vi "Channel Read Write.vi"(11 "plugin gRPC address":string="localhost:51930") -> ()   [LabVIEW 2021, in "CAN_Reader_NIXNET_Test_Helpers.lvlib"]
uses:
  CAN_Reader_NIXNET_Test_Helpers.lvlib
  <vilib>/CIF Foundation/CIF Core/CIFCore/Common/Typedef/gRPC Reported Plugin Status.ctl
  <vilib>/CIF Foundation/CIF Core/CIFCore/Common/Typedef/Plugin State.ctl
  <vilib>/CIF Foundation/CIF Core/CIFCore/Common/Typedef/Timing Statistics.ctl
  <vilib>/CIF Foundation/CIF Core/CIFCore/Common/Typedef/Timing Stats Base.ctl
  <vilib>/CIF Foundation/CIF Core/CIFCore/Common/Typedef/FIFO Statistics.ctl
  <vilib>/CIF Foundation/CIF Core/CIFCore/Common/Typedef/Simple Error.ctl
  <vilib>/CIF Foundation/CIF Core/CIFCore/Common/Typedef/Monitor Doubles.ctl
  <vilib>/CIF Foundation/CIF Core/CIFCore/Common/Typedef/Monitor U64.ctl
  <vilib>/CIF Foundation/CIF Core/CIFCore/Common/Typedef/Monitor I64.ctl
  <vilib>/CIF Foundation/CIF Channels Core/ChannelCommon/typedef/FIFO Header.ctl
  <vilib>/xnet/xnet.llb/XNET Frame CAN.ctl
  <vilib>/xnet/xnet.llb/XNET Frame Type CAN.ctl
  Common/Typedef/Channels.ctl
  <vilib>/CIF Foundation/CIF Core/CIFCore/Class/CIFCorePlugin.lvclass/CIFCorePlugin.ctl
  <vilib>/CIF Foundation/CIF Utilities/Statistics/I64/Stats_I64_CIF_U.lvclass/Stats_I64_CIF_U.ctl
  <vilib>/CIF Foundation/CIF XNET CAN RW/XNET CAN RW.lvclass
  C:/Program Files/National Instruments/LabVIEW 2021/vi.lib/CIF Foundation/CIF CAN RW Core/CAN_RW_CORE.lvclass
  <vilib>/CIF Foundation/CIF CAN RW Core/CAN_RW_CORE.lvclass/CAN_RW_CORE.ctl
  <vilib>/CIF Foundation/CIF PCAP Parse and Build/pcap_Parse_Build_CIF.lvclass/pcap_Parse_Build_CIF.ctl
  <vilib>/CIF Foundation/CIF Core/CIFCore/Class/Benchmarking/Benchmark FIFO Read.vi
  <vilib>/CIF Foundation/CIF XNET CAN RW/Utilities/Header Cluster to XNET CAN.vi
  <vilib>/CIF Foundation/CIF PCAP Parse and Build/Parse/Parse Packet Header.vi
  <vilib>/CIF Foundation/CIF PCAP Parse and Build/Parse/Unflatten Socket CAN Header.vi
  <vilib>/CIF Foundation/CIF PCAP Parse and Build/Utilities/Get Data Segment.vi
  <vilib>/CIF Foundation/CIF PCAP Parse and Build/Data Accessors/Read Offset.vi
  <vilib>/CIF Foundation/CIF CAN RW Core/Utilities/Filter Packets.vi
  <vilib>/CIF Foundation/CIF CAN RW Core/Accessors/Read pcap class.vi
  <vilib>/CIF Foundation/CIF CAN RW Core/Accessors/Write pcap class.vi
  <vilib>/CIF Foundation/CIF PCAP Parse and Build/Data Accessors/Write Offset.vi
  <vilib>/CIF Foundation/CIF Utilities/Statistics/I64/X1 minus X0.vi
  <vilib>/CIF Foundation/CIF Utilities/Time/System Time/Get System Time.vi
  <vilib>/CIF Foundation/CIF Utilities/Time/System Time/TAI Time to LabVIEW Time.vi
  <vilib>/CIF Foundation/CIF PCAP Parse and Build/Parse/Unflatten Packet Header.vi
  <vilib>/CIF Foundation/CIF Utilities/DataTypes/Flatten Unflatten/Unflatten U32.vi
  <vilib>/CIF Foundation/CIF PCAP Parse and Build/Utilities/Add Error.vi
  <vilib>/CIF Foundation/CIF Utilities/Statistics/I64/X1 minus X0.vi/dfabcf33-0dbc-4041-80a5-3dc0c86d2989.vi
  <vilib>/CIF Foundation/CIF Utilities/Errors/Append Error Location.vi
  <vilib>/CIF Foundation/CIF Utilities/Statistics/I64/X1 minus X0.vi/dfabcf33-0dbc-4041-80a5-3dc0c86d2989.vi/9eb60a9a-770f-4d2d-8b3f-8465c267ecc9.vi
  <vilib>/gRPC/LabVIEW gRPC Library/Client API/Close Client.vi
  <vilib>/CIF Foundation/CIF PCAP Parse and Build/pcap_Parse_Build_CIF.lvclass
  <vilib>/CIF Foundation/CIF Channels Core/CIFChannels/CIFChannels.lvclass
  <vilib>/CIF Foundation/CIF Core/CIFCore/Grpc/CIFCoreWrapper/CIFCoreWrapper.lvlib
  <vilib>/CIF Foundation/CIF Core/CIFCore/Class/CIFCorePlugin.lvclass
  Common/CAN_Reader_NIXNET_Common.lvlib
  Grpc/CAN_Reader_NIXNET_wrapper/CAN_Reader_NIXNET_Wrapper.lvlib
  <vilib>/CIF Foundation/CIF Utilities/DataTypes/DataTypes_CIF_U.lvlib
  <vilib>/CIF Foundation/CIF Utilities/Time/Time_CIF_U.lvlib
  <vilib>/CIF Foundation/CIF Core/CIFCore/Common/CIFCoreCommon.lvlib
  <vilib>/CIF Foundation/CIF Channels Core/ChannelCommon/ChannelCommon.lvlib
panel:
  out "x-y":i64 format="%.5e"
  out "Raw Bytes":string
  out "XNET CAN Data":T1[](array[typedef]) {"payload" format="%x"; "timestamp" format="%<%.7X\n%x>T"; "type" items=["CAN Data"=0, "CAN Remote"=1, "CAN Bus Error"=2, "CAN 2.0 Data"=8, "CAN FD Data"=16, "CAN FD+BRS Data"=24, "J1939 Data"=192, "Delay"=224, "Log Trigger"=225, "Start Trigger"=226]; "identifier" format="%x"}
  out "Header":T3
  out "Node Status":T4 {"Monitor Doubles"."4" format="%#_9g"; "Monitor Doubles"."3" format="%#_9g"; "Monitor Doubles"."2" format="%#_9g"; "Monitor Doubles"."1" format="%#_9g"; "Timing Statistics (us)"."Period"."Avg" format="%_6g"}
  in  "EXIT":bool
  in  "Unload":bool
  out "error out":errorcluster
  # "Update plugin gRPC address including gRPC port and run on same target as the plugin code. \nExit will stop this VI.\nUnload will stop this VI and unload the plugin."
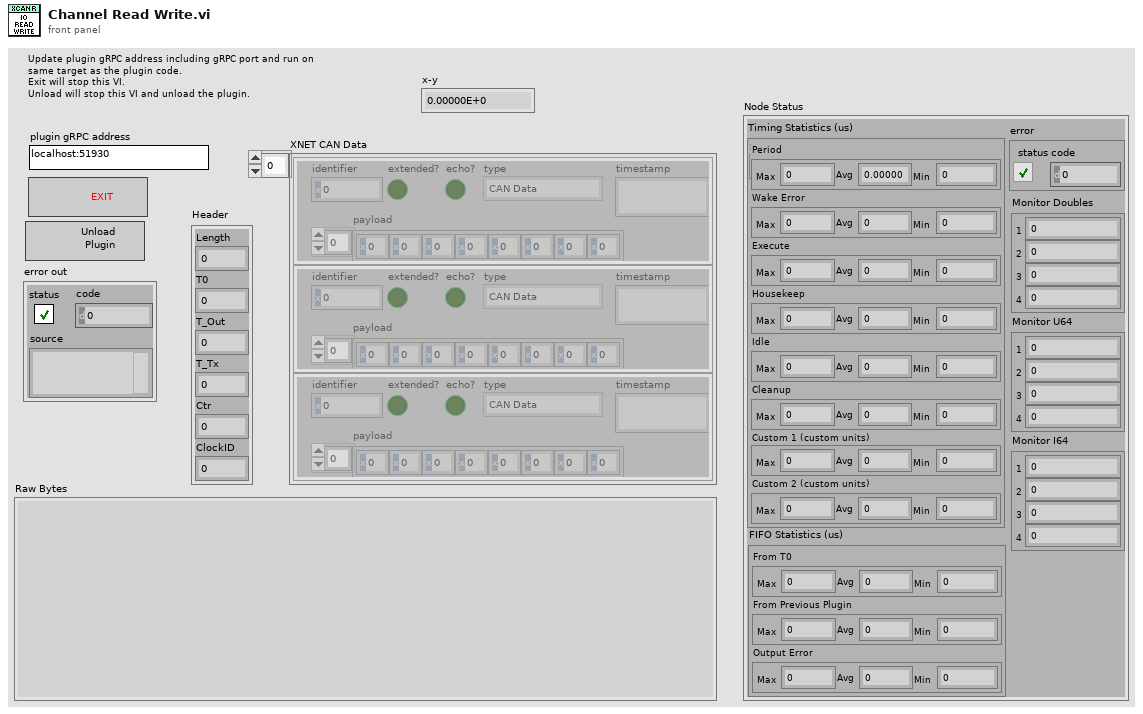
[diagram p1: front panel]
types:
  T1 = typedef "XNET Frame CAN.ctl" = cluster{"timestamp":timestamp, "payload":u8[], "identifier":u32, "type":T2, "extended?":bool, "echo?":bool}
  T2 = typedef "XNET Frame Type CAN.ctl" = u8
  T3 = typedef "ChannelCommon.lvlib/FIFO Header.ctl" = cluster{"Length":u64, "T0":i64, "T_Out":i64, "T_Tx":i64, "Ctr":u64, "ClockID":u8}
  T4 = typedef "CIFCoreCommon.lvlib/gRPC Reported Plugin Status.ctl" = cluster{"State":T5, "Timing Statistics (us)":T6, "FIFO Statistics (us)":T8, "error":T9, "Monitor Doubles":T10, "Monitor U64":T11, "Monitor I64":T12}
  T5 = typedef "CIFCoreCommon.lvlib/Plugin State.ctl" = enum32{"Null", "Creating", "Listening", "Running", "CleaningUp", "Destroying"}
  T6 = typedef "CIFCoreCommon.lvlib/Timing Statistics.ctl" = cluster{"Period":T7, "Wake Error":T7, "Execute":T7, "Housekeep":T7, "Idle":T7, "Cleanup":T7, "Custom 1 (custom units)":T7, "Custom 2 (custom units)":T7}
  T7 = typedef "CIFCoreCommon.lvlib/Timing Stats Base.ctl" = cluster{"Max":i64, "Avg":dbl, "Min":i64}
  T8 = typedef "CIFCoreCommon.lvlib/FIFO Statistics.ctl" = cluster{"From T0":T7, "From Previous Plugin":T7, "Output Error":T7}
  T9 = typedef "CIFCoreCommon.lvlib/Simple Error.ctl" = cluster{"status":bool, "code":i32}
  T10 = typedef "CIFCoreCommon.lvlib/Monitor Doubles.ctl" = cluster{"1":dbl, "2":dbl, "3":dbl, "4":dbl}
  T11 = typedef "CIFCoreCommon.lvlib/Monitor U64.ctl" = cluster{"1":u64, "2":u64, "3":u64, "4":u64}
  T12 = typedef "CIFCoreCommon.lvlib/Monitor I64.ctl" = cluster{"1":i64, "2":i64, "3":i64, "4":i64}
  T13 = typedef "grpc-lvsupport-release.lvlib/grpcId.ctl" = u64
  T14 = typedef "CIFCoreChannel_client.lvlib/cif_channelcore_Channel.ctl" = cluster{"name":string, "direction":T15, "type":string, "custom_config":u8[], "connected":bool, "connected_name":string, "forced":bool, "channel_pattern":T16}
  T15 = typedef "CIFCoreChannel_client.lvlib/cif_channelcore_Direction.ctl" = enum32{"PUBLISHER", "SUBSCRIBER"}
  T16 = typedef "CIFCoreChannel_client.lvlib/cif_channelcore_PATTERN.ctl" = enum32{"UNKNOWN", "TAG", "FIFO", "MULTIFIFO", "BACKPRESSUREFIFO"}
  T17 = typedef "CAN_Reader_NIXNET_Common.lvlib/Channels.ctl" = enum16{"CAN_Frames"}
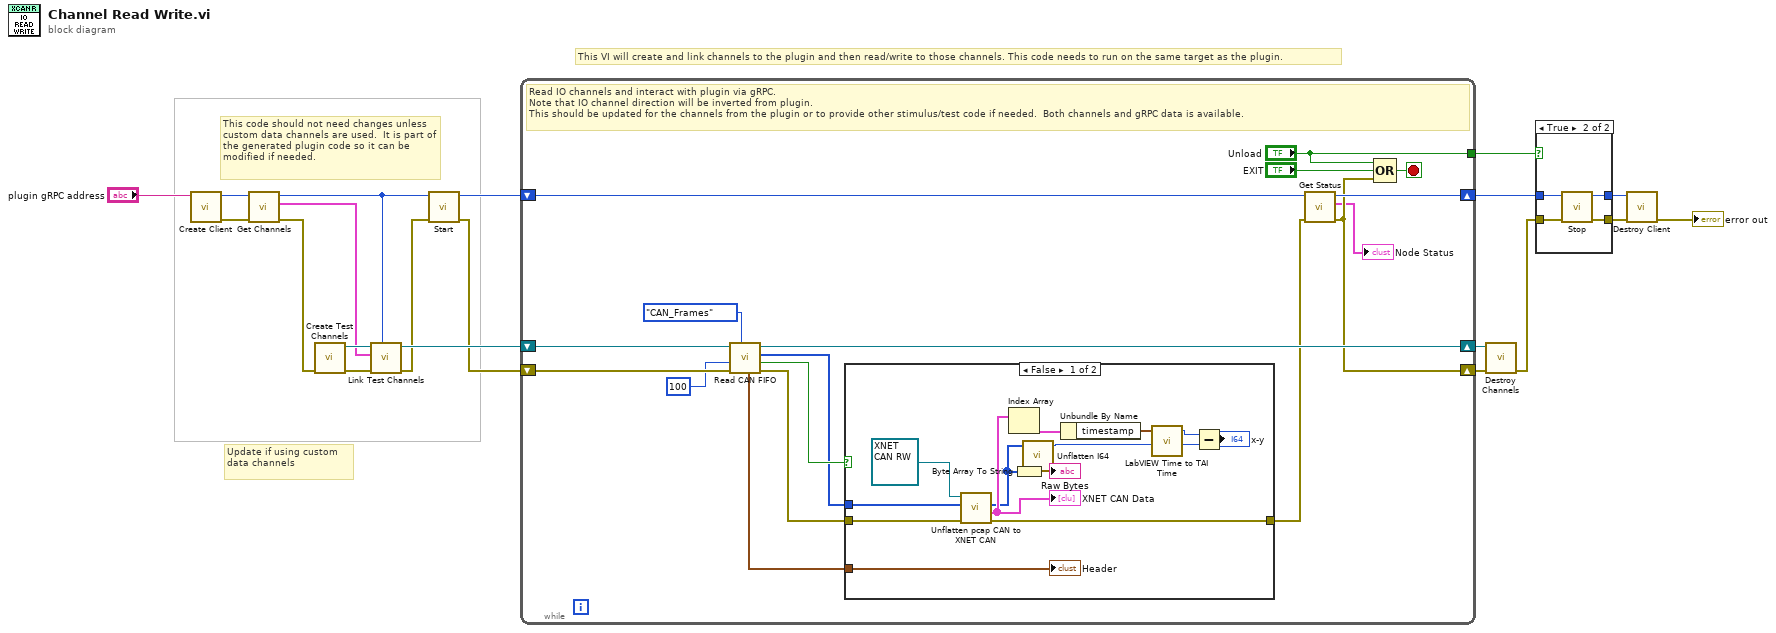
[diagram p0: block diagram]
diagram:
  # "Update if using custom data channels"
  # "This code should not need changes unless custom data channels are used.  It is part of the generated plugin code so it can be modified if needed."
  # "This VI will create and link channels to the plugin and then read/write to those channels. This code needs to run on the same target as the plugin."
  n1 = call "Create Client.vi"("address"="plugin gRPC address") -> ("error out"=w11:errorcluster, "gRPC ID Out"=w10:T13)  [unwired: 9 in]
  n2 = call <vilib>:"Get Channels.vi"("error in"=w11, "gRPC ID"=w10) -> ("error out"=w19:errorcluster, "Channels"=w15:T14[], "gRPC ID out"=w9:T13)  [unwired: 7 in]
  n3 = call "Create Test Channels.vi"("error in"=w19) -> ("error out"=w18:errorcluster, "CIFCorePlugin out"=w17:refnum<class "CIFCorePlugin.lvclass">)  [unwired: 9 in]
  n4 = call "Link Test Channels.vi"("gRPC ID in"=w9, "error in (no error)"=w18, "Channels"=w15, "CIFCorePlugin in"=w17) -> ("error out"=w7:errorcluster, "CIFCorePlugin out"=w16:refnum<class "CIFCorePlugin.lvclass">)  [unwired: 6 in]
  n5 = call <vilib>:"Start.vi"("error in"=w7, "gRPC ID"=w9) -> ("error out"=w6:errorcluster, "gRPC ID out"=w8:T13)  [unwired: 8 in]
  n6 = while {
    shift-right: [w35] -> w20
    shift-left: w16 -> [w28]
    shift-right: [w34] -> w14
    shift-left: w6 -> [w27]
    shift-right: [w36] -> w4
    shift-left: w8 -> [w37]
    tunnel: ["Unload"] -> w1
    stop <- w33 stop-if-true
    # "Read IO channels and interact with plugin via gRPC.\nNote that IO channel direction will be inverted from plugin.\nThis should be updated for the channels from the plugin or to provide other stimulus/test code if needed.  Both channels and gRPC data is available."
    n7 = call <vilib>:"Read CAN FIFO.vi"("Channel Index"=Channels."CAN_Frames" ("Channels"), "error in (no error)"=w27, "Timeout (ms)"=100, "CIFCorePlugin in"=w28) -> ("error out"=w22:errorcluster, "timed out?"=w24:bool, "Data"=w23:u8[], "CIFCorePlugin out"=w35:refnum<class "CIFCorePlugin.lvclass">, "Header"=w26:T3)  [unwired: 3 in]
    n8 = case shown="False" w24 {
      tunnel: w26 -> [w50 _]
      tunnel: w23 -> [w49 _]
      tunnel: w22 -> [w48 w51]
      tunnel: [w47 w51] -> w21
      frame False {
        n9 = call <vilib>:"Unflatten pcap CAN to XNET CAN.vi"("error in (no error)"=w48, "pcap CAN DATA in"=w49, "XNET_CAN_RW in"=refnum<class "XNET CAN RW.lvclass"> refnum) -> ("error out"=w47:errorcluster, "XNET CAN Data"=w44:T1[], "pcap CAN DATA out"=w42:u8[])  [unwired: 3 in, 3 out]
        "XNET CAN Data" <- w44
        n10 = Index Array(array=w44) -> (element=w43:T1)  [unwired: 1 in]
        n11 = Byte Array To String(unsigned byte array=w42) -> (string=→"Raw Bytes":string)
        n12 = call <vilib>:"Unflatten I64.vi"("Flat Data"=w42) -> ("I64"=w39:i64)  [unwired: 4 in]
        n13 = Unbundle By Name(w43) -> ("timestamp"=w41:timestamp)
        n14 = call <vilib>:"LabVIEW Time to TAI Time.vi"("LabVIEW Time (s)"=w41) -> ("TAI Time (ns)"=w40:i64)  [unwired: 4 in]
        n15 = Subtract(x=w40, y=w39) -> (x-y=→"x-y":i64)
        "Header" <- w50
      }
      frame True {
      }
    }
    n16 = call <vilib>:"Get Status.vi"("error in"=w21, "gRPC ID"=w37) -> ("error out"=w34:errorcluster, "Node Status"=→"Node Status":T4, "gRPC ID out"=w36:T13)  [unwired: 7 in]
    n17 = Compound Arithmetic op=OR("Unload", "EXIT", w34) -> (w33:bool)
  }
  n18 = call <vilib>:"Destroy Channels.vi"("error in (no error)"=w14, "CIFCorePlugin in"=w20) -> ("error out"=w5:errorcluster)  [unwired: 7 in, 2 out]
  n19 = case shown="True" w1 {
    tunnel: w5 -> [w52 w57]
    tunnel: w4 -> [w53 w56]
    tunnel: [w53 w55] -> w3
    tunnel: [w52 w54] -> w2
    frame False {
    }
    frame True {
      n20 = call <vilib>:"Stop.vi"("error in"=w57, "gRPC ID"=w56) -> ("error out"=w54:errorcluster, "gRPC ID out"=w55:T13)  [unwired: 8 in]
    }
  }
  n21 = call "Destroy Client.vi"("error in"=w2, "gRPC ID"=w3) -> ("error out"=→"error out":errorcluster)  [unwired: 9 in]
